vi "ctrlBoolLeft (SubVI).vi"(8 "error in":errorcluster, 10 "Position:Left":i32, 11 "Array":refnum<vi>[](array[refnum])) -> (0 "error out":errorcluster)   [LabVIEW 2017]
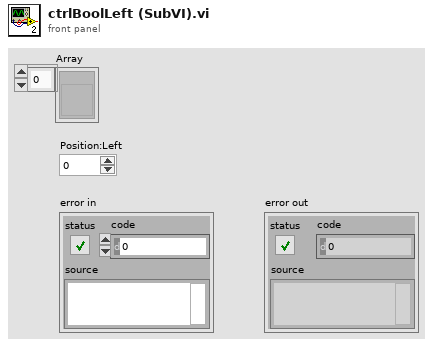
[diagram p1: front panel]
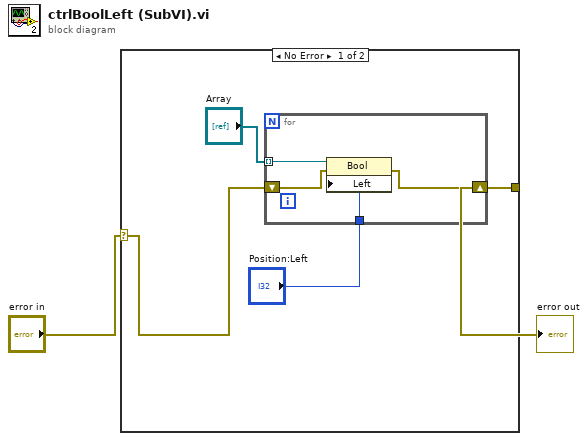
[diagram p0: block diagram]
diagram:
  n1 = case shown="No Error" "error in" {
    selector: "error in" -> [w4 w11]
    tunnel: [w5 w11] -> w2
    frame No Error {
      n2 = for {
        tunnel: "Array" -> [w10] mode=indexing
        shift-right: [w9] -> w5
        shift-left: w4 -> [w8]
        tunnel: "Position:Left" -> [w7]
        n3 = property on="Property Node" class="Bool"(reference=w10, error in=w8, "Left"=w7) -> (error out=w9:errorcluster)  [unwired: 1 out]
      }
    }
    frame Error {
    }
  }
  "error out" <- w2
